vi "OwnOop20261013_CreateChildV4.vi"() -> ()   [LabVIEW 2024]
uses:
  <resource>/Framework/Providers/AddClass/Add Class.lvlib
panel:
  out "error out":errorcluster caption="错误输出"
  in  "Parent Interfaces":refnum<vi>[](array[refnum])
  in  "New Class Owner":refnum<vi>
  in  "Class Path":path
  in  "Parent Path":path
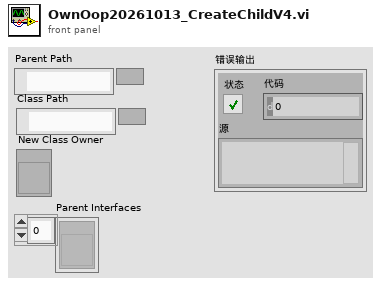
[diagram p1: front panel]
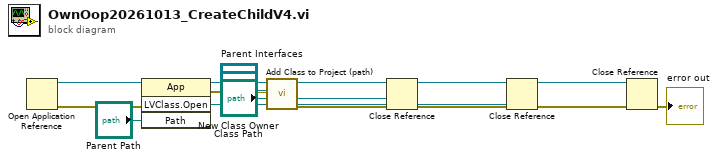
[diagram p0: block diagram]
diagram:
  n1 = Open Application Reference() -> (0:w11:errorcluster, 3:w13:refnum<vi>)  [unwired: 4 in]
  n2 = invoke class="App" method="LVClass.Open"(reference=w13, error in=w11, "Path"="Parent Path") -> (error out=w6:errorcluster, "LVClass.Open"=w7:refnum<vi>)  [unwired: 1 in, 2 out]
  n3 = call <resource>:"Add Class to Project (path).vi"("Parent Class"=w7, "Application"=w13, "error in"=w6, "Class Path"="Class Path", "New Class Owner"="New Class Owner", "Parent Interfaces"="Parent Interfaces") -> ("error out"=w4:errorcluster, "Class"=w5:refnum<vi>)  [unwired: 4 in]
  n4 = Close Reference(reference=w5, error in (no error)=w4) -> (error out=w3:errorcluster)
  n5 = Close Reference(reference=w7, error in (no error)=w3) -> (error out=w2:errorcluster)
  n6 = Close Reference(reference=w13, error in (no error)=w2) -> (error out=→"error out":errorcluster)
